vi "usbpt104UnitInfo.vi"(8 "error in (no error)":errorcluster, 11 "handle in":i16=16384) -> (0 "error out":errorcluster, 2 "Unit Info":T1, 3 "handle out":i16=16384)   [LabVIEW 2010]
doc: "Returns Driver and Unit Information"
uses:
  UsbPT104.dll
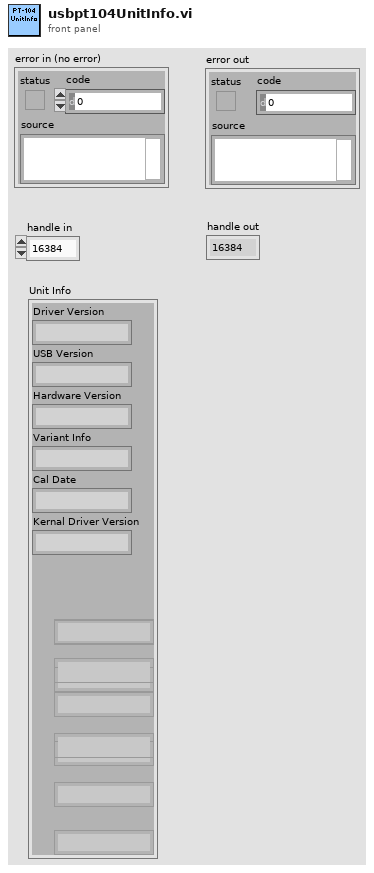
[diagram p1: front panel]
types:
  T1 = cluster{"Driver Version":string, "USB Version":string, "Hardware Version":string, "Variant Info":string, "Cal Date":string, "Kernal Driver Version":string, "NA":string, "NA 2":string, "NA":string, "NA 3":string, "NA 4":string, "NA 5":string, "NA 6":string, "NA 7":string, "NA 8":string}
  T2 = cluster{"status":bool, "code":u32, "source":string}
  T3 = cluster{"[0]":string, "[1]":string, "[2]":string, "[3]":string, "[4]":string, "[5]":string, "[6]":string, "[7]":string, "[8]":string, "[9]":string, "[10]":string, "[11]":string, "[12]":string, "[13]":string, "[14]":string}
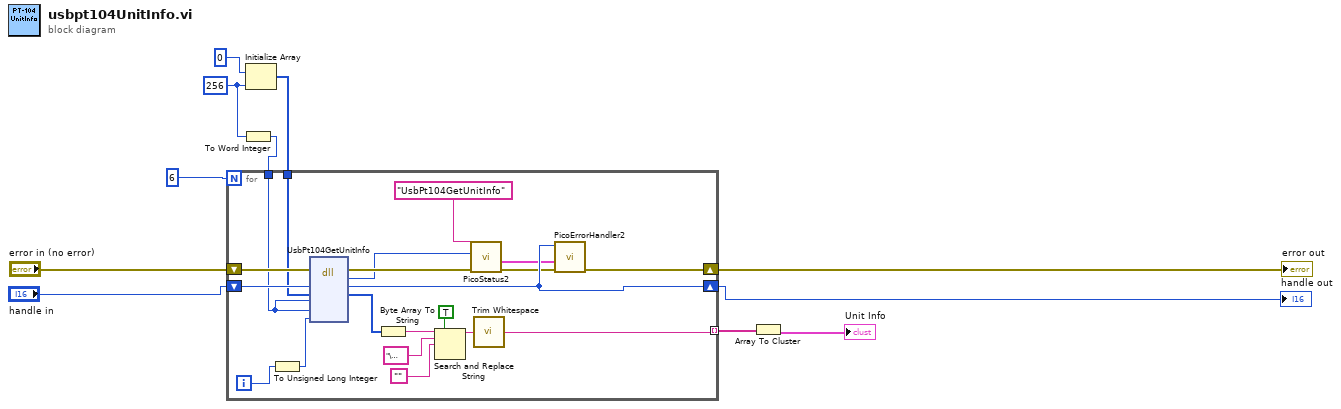
[diagram p0: block diagram]
diagram:
  w5 = 256 ("dimension size")
  n1 = To Word Integer(number=w5) -> (16bit integer=w4:i16)
  n2 = Initialize Array(u8 0 ("element"), w5) -> (w11:u8[])
  n3 = for {
    N: 6 -> [_]
    tunnel: [w18] -> w8 mode=indexing
    tunnel: w11 -> [w25]
    shift-right: [w19] -> w2
    shift-left: "handle in" -> [w27]
    shift-right: [w20] -> w3
    shift-left: "error in (no error)" -> [w26]
    tunnel: w4 -> [w17]
    i -> [w21]
    n4 = To Unsigned Long Integer(number=w21) -> (unsigned 32bit integer=w22:u32)
    n5 = dll-call lib="UsbPT104.dll" fn="UsbPt104GetUnitInfo"(error in=w26, "handle"=w27, "String"=w25, "StringLength"=w17, "requiredSize"=w17, "info"=w22) -> (error out=w14:errorcluster, "PICO_STATUS"=w13:u32, "handle"=w19:i16, "String"=w24:u8[])  [unwired: 5 in, 1 out]
    n6 = Byte Array To String(unsigned byte array=w24) -> (string=w23:string)
    n7 = Search and Replace String(replace all?=TRUE ("replace all? (F)"), input string=w23, search string="\u0000", replace string="") -> (result string=w28:string)  [unwired: 4 in, 3 out]
    n8 = call "PicoStatus2.vi"("PICO source"="UsbPt104GetUnitInfo" ("source"), "Error in"=w14, "PICO STATUS"=w13) -> ("error out"=w16:errorcluster, "PICO_STATUS out"=w15:T2)  [unwired: 5 in]
    n9 = call <vilib>:"Trim Whitespace.vi"("string"=w28) -> ("trimmed string"=w18:string)  [unwired: 1 in]
    n10 = call "PicoErrorHandler2.vi"("error in (no error)"=w16, "PICO_STATUS in"=w15, "handle In"=w19) -> ("error out"=w20:errorcluster)  [unwired: 8 in]
  }
  "error out" <- w3
  "handle out" <- w2
  n11 = Array To Cluster(array=w8) -> (cluster=→"Unit Info":T3)
